vi "Write Log Line.vi"(10 "log line":string, 11 "string handler in":refnum<class "String Handler.lvclass">) -> (0 "error out":errorcluster, 3 "string handler out":refnum<class "String Handler.lvclass">)   [LabVIEW 2018, in "GLog.lvlib" / "String Handler.lvclass"]
uses:
  String Handler.lvclass
  C:/Users/Colin/Documents/software_projects/labview/glog/src/api/extension/formatting_handler_interface/Formatting Handler.lvclass
  extension/formatting_handler_interface/Formatting Handler.lvclass/Formatting Handler.ctl
  UI Updater/UI Updater.lvlib
  extension/formatting_handler_interface/Formatting Handler.lvclass
panel:
  # "Connector Pane"
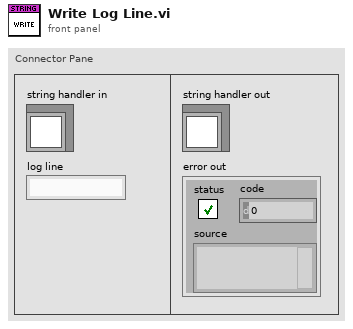
[diagram p1: front panel]
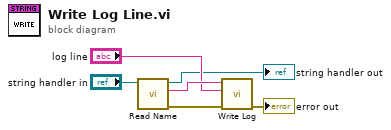
[diagram p0: block diagram]
diagram:
  n1 = call "Read Name.vi"("Formatting Handler in"="string handler in") -> ("error out"=w2:errorcluster, "Name"=w5:string, "Formatting Handler out"=→"string handler out":refnum<class "String Handler.lvclass">)  [unwired: 8 in]
  n2 = call "Write Log.vi"("error in (no error)"=w2, "formatted record"="log line", "handler name"=w5) -> ("error out"=→"error out":errorcluster)  [unwired: 8 in]
